vi "InitializeDotsByIndex.vi"(8 "error in (no error)":errorcluster, 10 "Dots":string[](array[string]), 11 "Setting Database in":refnum<class "Setting Database.lvclass">) -> (0 "error out":errorcluster, 3 "Setting Database out":refnum<class "Setting Database.lvclass">)   [LabVIEW 2019, in "Setting Database.lvclass"]
uses:
  Setting Database.lvclass
  Dot Settings/Dot Settings.lvclass
  C:/Users/Albro/Documents/GitHub/AFM-Lithography/lvsrc/Classes/Settings/ObjectSettings/ObjectSettings.lvclass
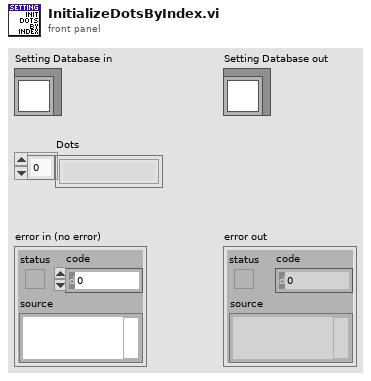
[diagram p1: front panel]
types:
  T1 = cluster{"Path":string, "Funnel":string, "Rectangle":string, "Dot":string}
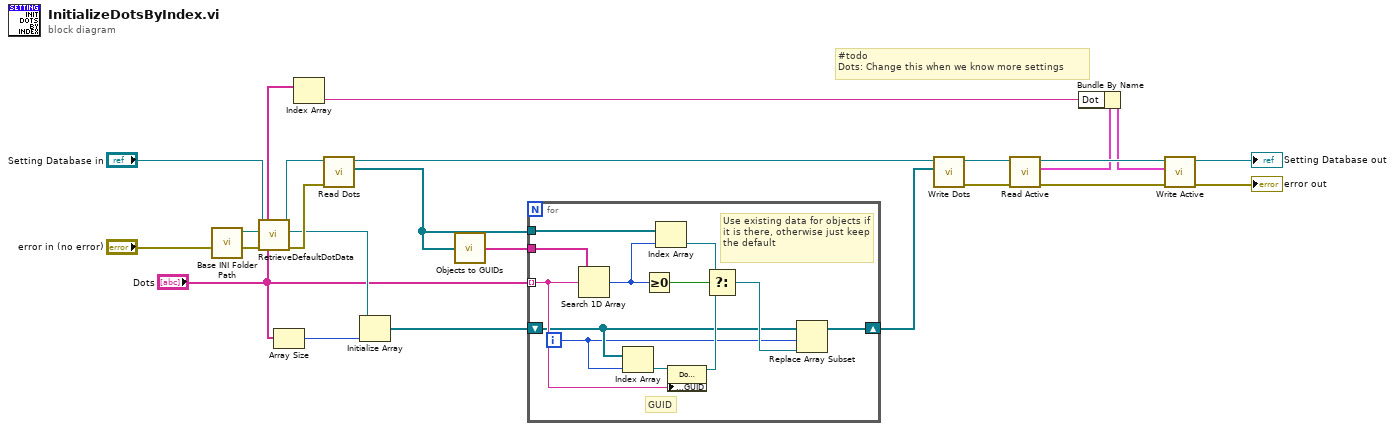
[diagram p0: block diagram]
diagram:
  # "#todo\nDots: Change this when we know more settings"
  n1 = call "Base INI Folder Path.vi"() -> ("Base Path"=w11:path)  [unwired: 11 in]
  n2 = call "RetrieveDefaultDotData.vi"("error in (no error)"="error in (no error)", "Path"=w11, "Setting Database In"="Setting Database in") -> ("error out"=w13:errorcluster, "Dot Settings out"=w8:refnum<class "Dot Settings.lvclass">, "Setting Database Out"=w9:refnum<class "Setting Database.lvclass">)  [unwired: 6 in]
  n3 = Array Size(array="Dots") -> (size(s)=w7:i32)
  n4 = Index Array(array="Dots") -> (element=w1:string)  [unwired: 1 in]
  n5 = call "Read Dots.vi"("error in (no error)"=w13, "Setting Database in"=w9) -> ("Dots"=w6:refnum<class "Dot Settings.lvclass">[], "Setting Database out"=w14:refnum<class "Setting Database.lvclass">)  [unwired: 7 in, 1 out]
  n6 = Initialize Array(w8, w7) -> (w4:refnum<class "Dot Settings.lvclass">[])
  n7 = call "Objects to GUIDs.vi"("Objects"=w6) -> ("GUIDs"=w5:string[])  [unwired: 3 in, 1 out]
  n8 = for {
    tunnel: w6 -> [w32]
    shift-right: [w34] -> w3
    shift-left: w4 -> [w24]
    tunnel: w5 -> [w31]
    tunnel: "Dots" -> [w29] mode=indexing
    i -> [w23]
    # "GUID"
    # "Use existing data for objects if it is there, otherwise just keep the default"
    n9 = Search 1D Array(1D array=w31, element=w29) -> (index of element=w33:i32)  [unwired: 1 in]
    n10 = Index Array(array=w24, index=w23) -> (element=w30:refnum<class "Dot Settings.lvclass">)
    n11 = Greater Or Equal To 0?(x=w33) -> (x >= 0?=w28:bool)
    n12 = Index Array(array=w32, index=w33) -> (element=w27:refnum<class "Dot Settings.lvclass">)
    n13 = property class="Dot Settings.lvclass"(reference=w30, "Accessors:GUID"=w29) -> (reference out=w25:refnum<class "Dot Settings.lvclass">)  [unwired: 1 in, 1 out]
    n14 = Select(t=w27, s=w28, f=w25) -> (s? t:f=w26:refnum<class "Dot Settings.lvclass">)
    n15 = Replace Array Subset(array=w24, new element=w26, index=w23) -> (w34:refnum<class "Dot Settings.lvclass">[])
  }
  n16 = call "Write Dots.vi"("Dots"=w3, "Setting Database in"=w14) -> ("error out"=w16:errorcluster, "Setting Database out"=w21:refnum<class "Setting Database.lvclass">)  [unwired: 8 in]
  n17 = call "Read Active.vi"("error in (no error)"=w16, "Setting Database in"=w21) -> ("error out"=w17:errorcluster, "Active"=w19:T1, "Setting Database out"=w22:refnum<class "Setting Database.lvclass">)  [unwired: 7 in]
  n18 = Bundle By Name(cluster=w19, "Dot"=w1) -> (w18:T1)
  n19 = call "Write Active.vi"("error in (no error)"=w17, "Active"=w18, "Setting Database in"=w22) -> ("error out"=→"error out":errorcluster, "Setting Database out"=→"Setting Database out":refnum<class "Setting Database.lvclass">)  [unwired: 7 in]
